vi "State Machine User Manager.vi"() -> ()   [LabVIEW 2024]
doc: "This VI shows how to implement a state machine based, stand-alone user manager using the Easy User Manager package."
uses:
  EasyUserManager/EasyUserManager.lvclass
  <vilib>/regexp/Match Regular Expression.xnode
  Type Definitions/States.ctl
  Type Definitions/Data.ctl
panel:
  in  "Main Tab":T1(tab)=enum."Execution"
  out "Current User":string
  in  "Fill LoginName/Group from Lists":bool=TRUE
  in  "Groups":i32(listbox)=-1
  in  "Tab Control":T2(tab)
  in  "Create Group Button":bool
  in  "Group Name (Create/Delete)":string caption="Group Name"
  in  "Delete Group Button":bool
  in  "Create User Button":bool
  in  "LoginName (Create/Delete)":string caption="LoginName"
  in  "Password (Create)":string caption="Password (only needed for creating)"
  in  "Delete User Button":bool
  in  "New Privilege Value (User Parameters)":bool caption="New Value"
  in  "Privilege (User Configuration)":string caption="Privilege"
  in  "Set Privilege (User Parameters)":bool
  in  "Password (Parameters)":string caption="Password"
  in  "Set Password Button":bool
  in  "Set Full Name (User Parameters)":bool
  in  "Full Name (User Parameters)":string caption="Full Name"
  in  "LoginName (Configuration)":string caption="LoginName"
  in  "Add User to Group Button":bool
  in  "LoginName (Add/Rem User to Group)":string caption="LoginName (User)"
  in  "Group Name (Add/Rem User to Group)":string caption="Group Name"
  in  "Remove User from Group":bool
  in  "Set Group Privilege":bool
  in  "Privilege (Group)":string caption="Privilege"
  in  "New Privilege Value (Group)":bool caption="New Value"
  out "Group Exists Indicator":bool
  out "User Exists Indicator":bool
  in  "Group Exists":bool
  in  "Password (Validation)":string caption="Password"
  in  "LoginName (Validation)":string caption="LoginName"
  in  "Privilege (Validation)":string caption="Privilege"
  in  "Validate Password":bool
  out "Password OK":bool
  in  "Check Privilege":bool
  out "Has privilege":bool
  in  "User Exists":bool
  in  "Users (Groups)":i32(listbox)=-1
  in  "TestStand UI Application Manager":refnum<k7>(container)
  # "Logging in..."
  # "Shutting down..."
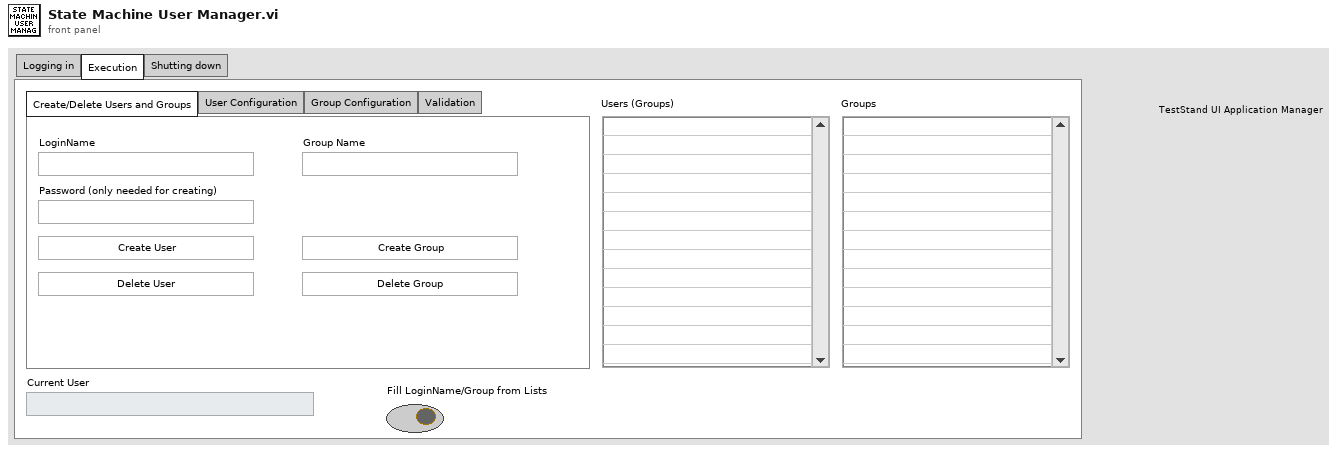
[diagram p1: front panel]
types:
  T1 = enum32{"Logging in", "Execution", "Shutting down"}
  T2 = enum32{"Create/Delete Users and Groups", "User Configuration", "Group Configuration", "Validation"}
  T3 = typedef "Data.ctl" = cluster{"Application Manager":refnum<k7>, "EasyUserManager":refnum<class "EasyUserManager.lvclass">}
  T4 = typedef "States.ctl" = enum16{"Initialize", "Start TS Application", "Wait for Login", "Check User Privilege", "Update User/Group Lists", "Idle", "Error", "Wrong Privileges", "Exit", "Wait for Shutdown", "Pre-Init Check", "Shutdown TS Application"}
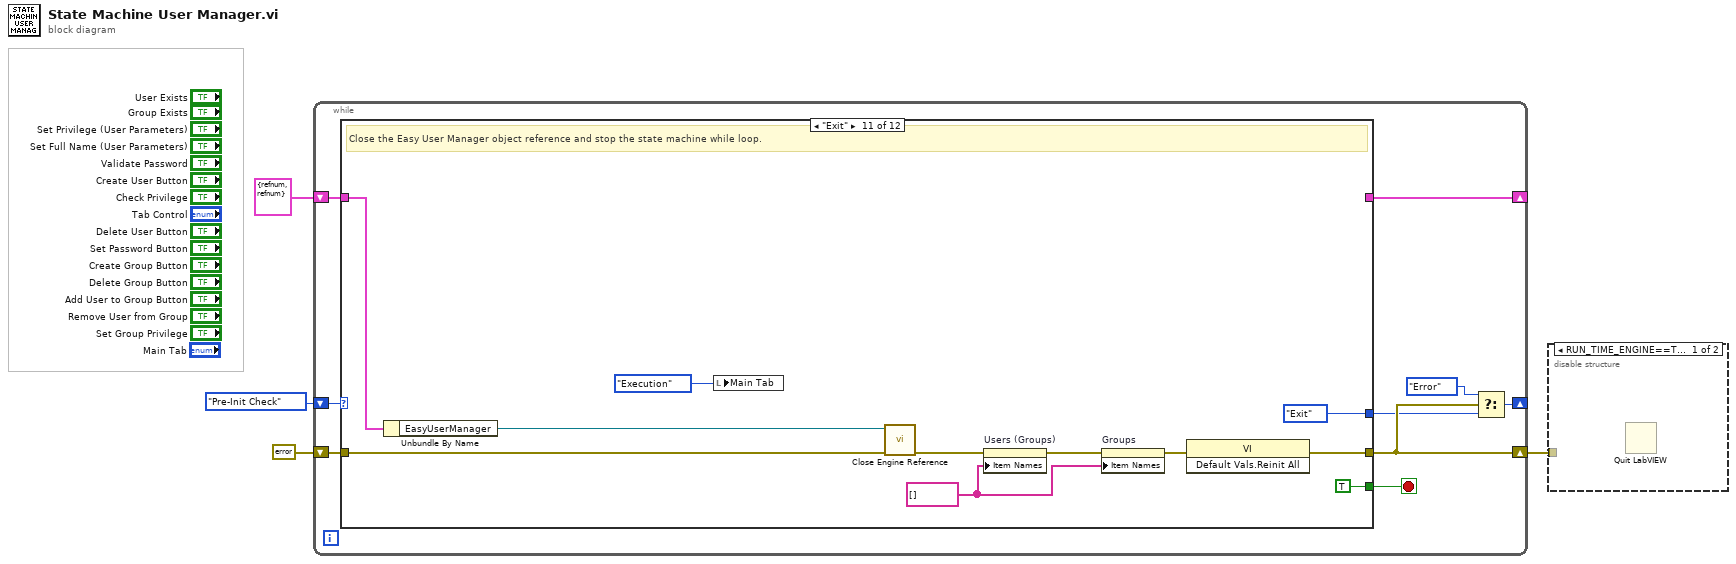
[diagram p0: block diagram]
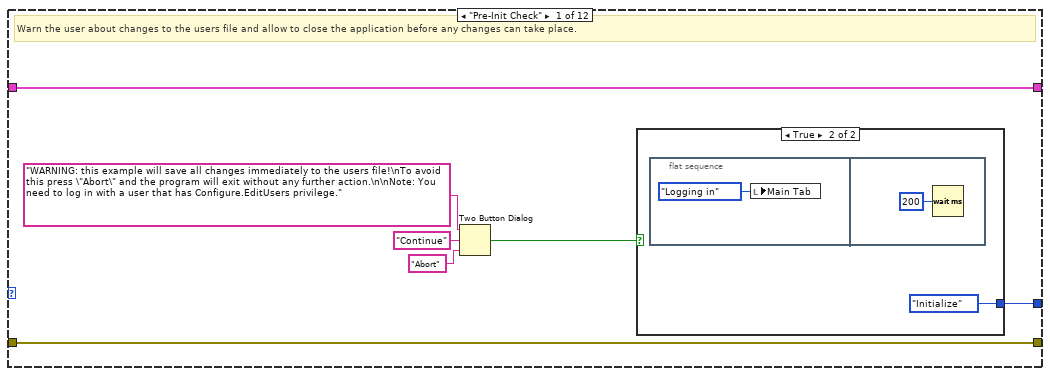
[diagram p3: hidden frame]
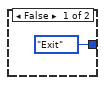
[diagram p4: hidden frame]
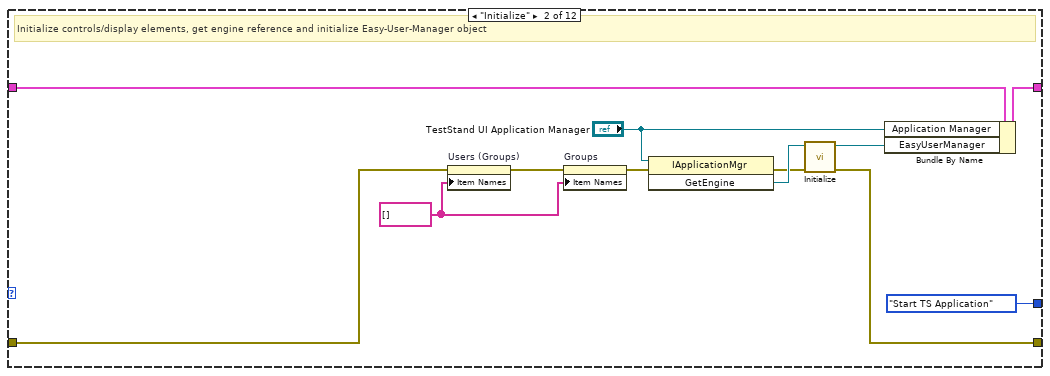
[diagram p5: hidden frame]
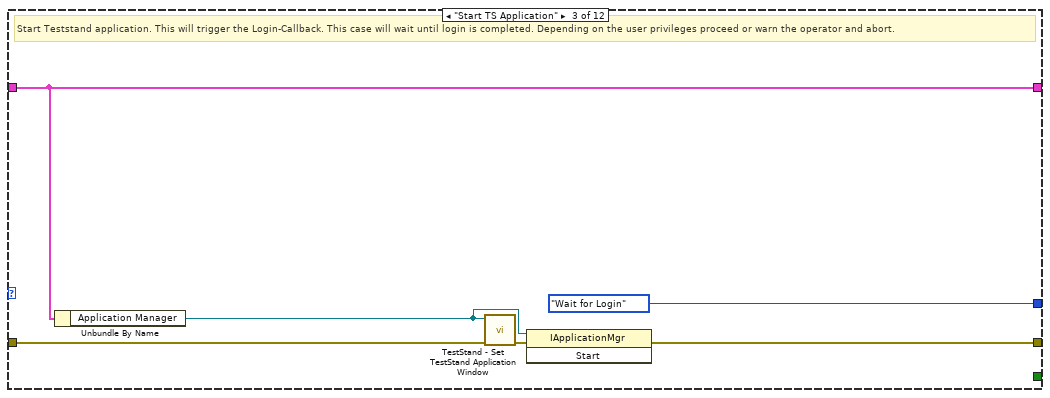
[diagram p6: hidden frame]
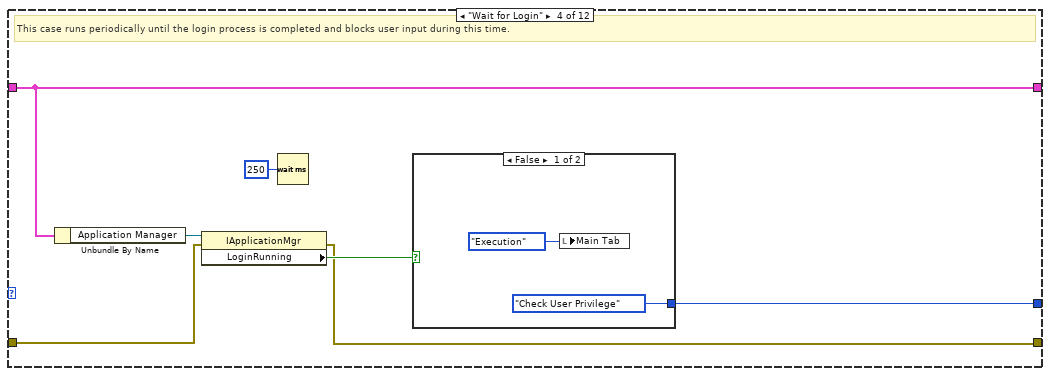
[diagram p7: hidden frame]
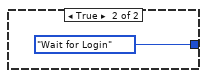
[diagram p8: hidden frame]
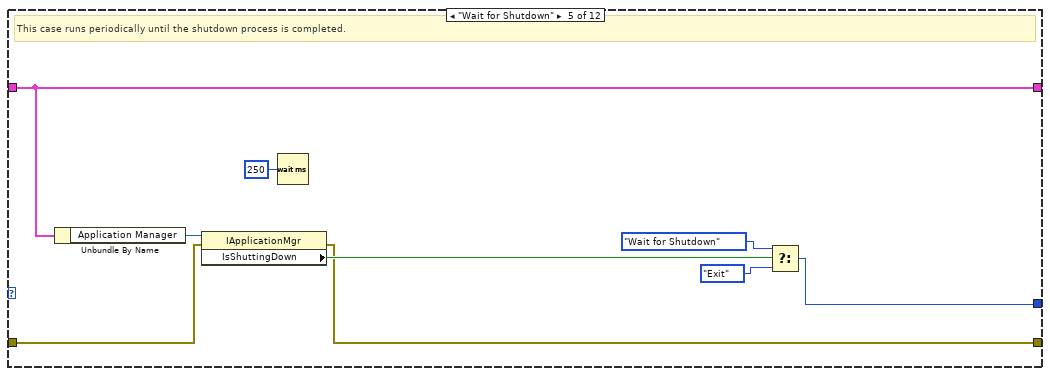
[diagram p9: hidden frame]
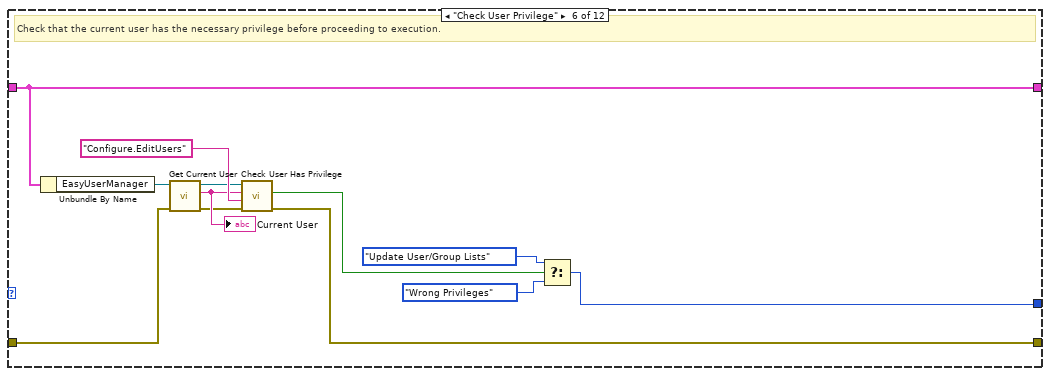
[diagram p10: hidden frame]
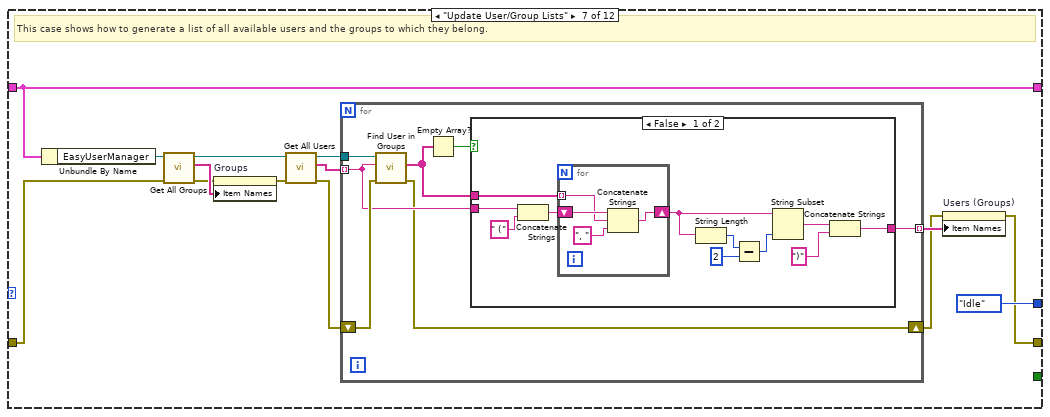
[diagram p11: hidden frame]
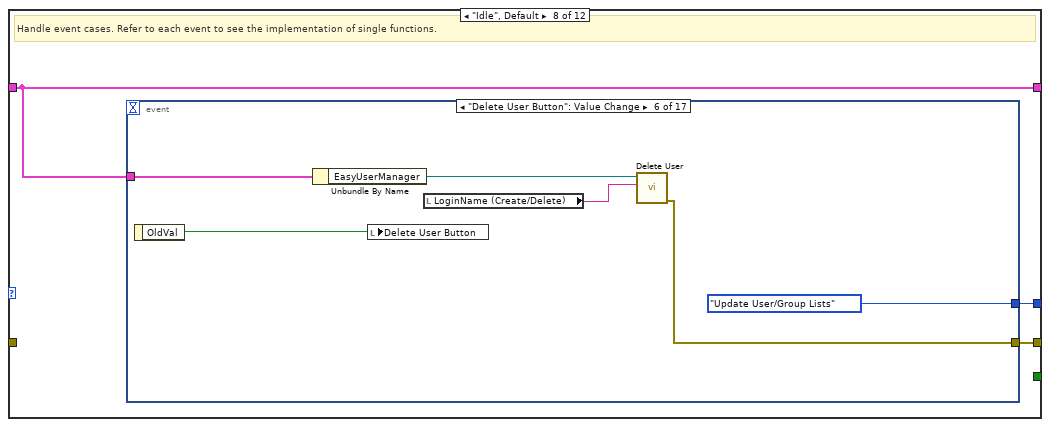
[diagram p13: hidden frame]
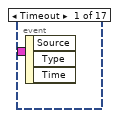
[diagram p14: hidden frame]
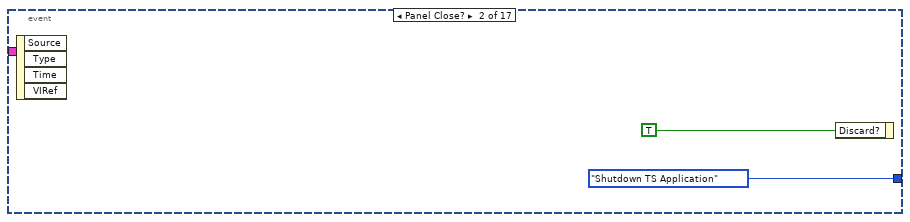
[diagram p15: hidden frame]
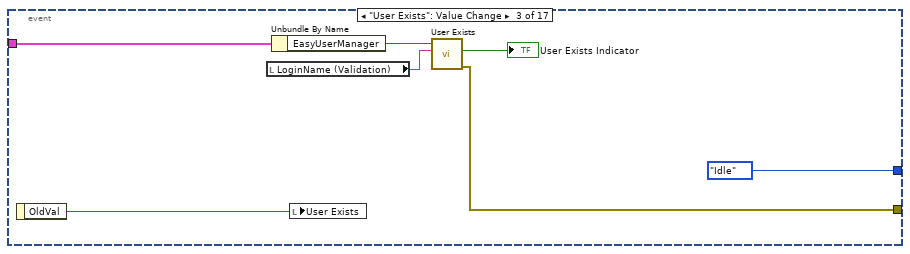
[diagram p16: hidden frame]
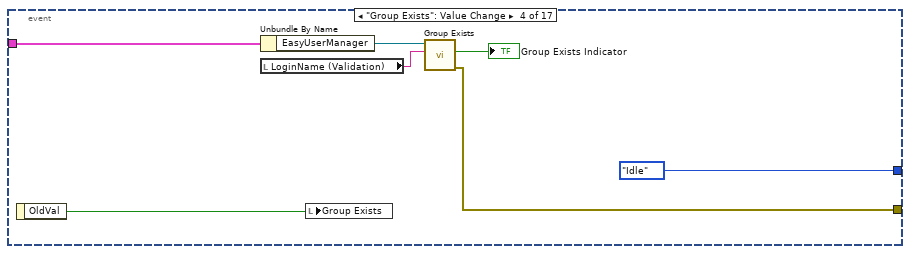
[diagram p17: hidden frame]
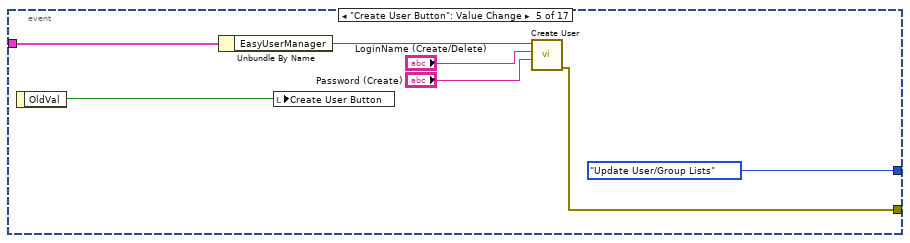
[diagram p18: hidden frame]
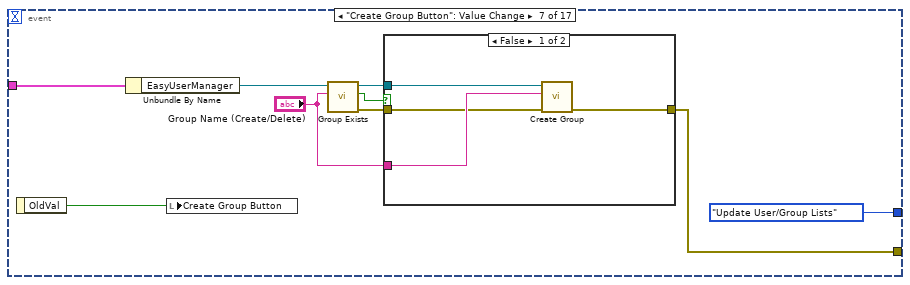
[diagram p19: hidden frame]
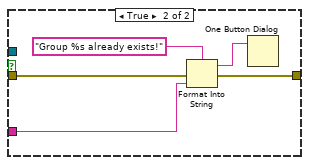
[diagram p20: hidden frame]
diagram:
  n1 = while {
    shift-right: [w6] -> _
    shift-left: States."Pre-Init Check" ("State") -> [w13]
    shift-right: [w5] -> _
    shift-left: T3 {"Application Manager"=refnum, "EasyUserManager"=refnum} ("Data") -> [w11]
    shift-right: [w9] -> w1
    shift-left: errorcluster {"status"=FALSE, "code"=0, "source"=""} ("error constant") -> [w10]
    stop <- w12 stop-if-true
    n2 = case shown="\"Exit\"" w13 {
      tunnel: [_ _ _ _ _ _ _ _ _ _ TRUE _] -> w12
      tunnel: w11 -> [w20 w35 w42 w49 w61 w69 w81 w112 w361 w368 w378 w382]
      tunnel: w10 -> [w16 w25 w37 w46 w58 w64 w74 _ w362 _ w375 w383]
      tunnel: [w16 w26 w38 w43 w53 w68 w82 w111 w358 _ w369 w380] -> w9
      tunnel: [w15 States."Start TS Application" ("State") States."Wait for Login" ("State") w44 w55 w67 States."Idle" ("State") w113 States."Shutdown TS Application" ("State") States."Shutdown TS Application" ("State") States."Exit" ("State") States."Wait for Shutdown" ("State")] -> w7
      tunnel: [w20 w33 w42 w49 w61 w69 w81 w112 w361 w368 _ w382] -> w5
      frame "Pre-Init Check" {
        # "Warn the user about changes to the users file and allow to close the application before any changes can take place."
        n3 = Two Button Dialog(message="WARNING: this example will save all changes immediately to the users file!\nTo avoid this press \"Abort\" and the program will exit without any further action.\n\nNote: You need to log in with a user that has Configure.EditUsers privilege.", 1:"Abort" ("F button name (\"Cancel\")"), 2:"Continue" ("T button name (\"OK\")")) -> (T button?=w14:bool)
        n4 = case shown="True" w14 {
          tunnel: [States."Exit" ("f") States."Initialize" ("State")] -> w15
          frame False {
          }
          frame True {
            n5 = flat-sequence {
              frame #0 {
                n6 = local write "Main Tab"(T1."Logging in" ("Value")) -> ()
              }
              frame #1 {
                n7 = Wait (ms)(milliseconds to wait=u32 200) -> ()  [unwired: 1 out]
              }
            }
          }
        }
      }
      frame "Initialize" {
        w27 = string[] []
        # "Initialize controls/display elements, get engine reference and initialize Easy-User-Manager object"
        n8 = property on="Users (Groups)" class="LstBox (strict)"(error in=w25, "Item Names"=w27) -> (error out=w29:errorcluster)  [unwired: 1 in, 1 out]
        n9 = property on="Groups" class="LstBox (strict)"(error in=w29, "Item Names"=w27) -> (error out=w28:errorcluster)  [unwired: 1 in, 1 out]
        n10 = invoke class="IApplicationMgr" method="GetEngine"(reference="TestStand UI Application Manager", error in=w28) -> (error out=w30:errorcluster, "GetEngine"=w32:refnum<k7>)  [unwired: 1 in, 1 out]
        n11 = call "Initialize.vi"("error in (no error)"=w30, "Engine Reference"=w32) -> ("error out"=w26:errorcluster, "EasyUserManager out"=w31:refnum<class "EasyUserManager.lvclass">)  [unwired: 4 in]
        n12 = Bundle By Name(cluster=w35, "Application Manager"="TestStand UI Application Manager", "EasyUserManager"=w31) -> (w33:T3)
      }
      frame "Start TS Application" {
        # "Start Teststand application. This will trigger the Login-Callback. This case will wait until login is completed. Depending on the user privileges proceed or warn the operator and abort."
        n13 = Unbundle By Name(w42) -> ("Application Manager"=w40:refnum<k7>)
        n14 = call <vilib>:"TestStand - Set TestStand Application Window.vi"("error in (no error)"=w37, "Application Manager"=w40) -> ("error out"=w41:errorcluster)  [unwired: 9 in]
        n15 = invoke class="IApplicationMgr" method="Start"(reference=w40, error in=w41) -> (error out=w38:errorcluster)  [unwired: 1 in, 2 out]
      }
      frame "Wait for Login" {
        # "This case runs periodically until the login process is completed and blocks user input during this time."
        n16 = Unbundle By Name(w49) -> ("Application Manager"=w48:refnum<k7>)
        n17 = property class="IApplicationMgr"(reference=w48, error in=w46) -> (error out=w43:errorcluster, "LoginRunning"=w45:bool)  [unwired: 1 out]
        n18 = Wait (ms)(milliseconds to wait=u32 250) -> ()  [unwired: 1 out]
        n19 = case shown="False" w45 {
          tunnel: [States."Check User Privilege" ("f") States."Wait for Login" ("State")] -> w44
          frame False {
            n20 = local write "Main Tab"(T1."Execution" ("Value")) -> ()
          }
          frame True {
          }
        }
      }
      frame "Wait for Shutdown" {
        # "This case runs periodically until the shutdown process is completed."
        n21 = Unbundle By Name(w61) -> ("Application Manager"=w60:refnum<k7>)
        n22 = property class="IApplicationMgr"(reference=w60, error in=w58) -> (error out=w53:errorcluster, "IsShuttingDown"=w57:bool)  [unwired: 1 out]
        n23 = Wait (ms)(milliseconds to wait=u32 250) -> ()  [unwired: 1 out]
        n24 = Select(t=States."Wait for Shutdown" ("f"), s=w57, f=States."Exit") -> (s? t:f=w55:T4)
      }
      frame "Check User Privilege" {
        # "Check that the current user has the necessary privilege before proceeding to execution."
        n25 = Unbundle By Name(w69) -> ("EasyUserManager"=w66:refnum<class "EasyUserManager.lvclass">)
        n26 = call "Get Current User.vi"("error in (no error)"=w64, "EasyUserManager in"=w66) -> ("error out"=w62:errorcluster, "LoginName"=w63:string, "EasyUserManager out"=w65:refnum<class "EasyUserManager.lvclass">)  [unwired: 3 in]
        "Current User" <- w63
        n27 = call "Check User Has Privilege.vi"("error in (no error)"=w62, "Privilege"="Configure.EditUsers", "LoginName"=w63, "EasyUserManager in"=w65) -> ("error out"=w68:errorcluster, "User Has Privilege"=w73:bool)  [unwired: 1 in, 1 out]
        n28 = Select(t=States."Update User/Group Lists" ("State"), s=w73, f=States."Wrong Privileges") -> (s? t:f=w67:T4)
      }
      frame "Update User/Group Lists" {
        # "This case shows how to generate a list of all available users and the groups to which they belong."
        n29 = Unbundle By Name(w81) -> ("EasyUserManager"=w79:refnum<class "EasyUserManager.lvclass">)
        n30 = call "Get All Groups.vi"("error in (no error)"=w74, "EasyUserManager in"=w79) -> ("error out"=w76:errorcluster, "Groups"=w77:string[], "EasyUserManager out"=w78:refnum<class "EasyUserManager.lvclass">)  [unwired: 3 in]
        n31 = property on="Groups" class="LstBox (strict)"(error in=w76, "Item Names"=w77) -> (error out=w75:errorcluster)  [unwired: 1 in, 1 out]
        n32 = call "Get All Users.vi"("error in (no error)"=w75, "EasyUserManager in"=w78) -> ("error out"=w86:errorcluster, "Users"=w85:string[], "EasyUserManager out"=w80:refnum<class "EasyUserManager.lvclass">)  [unwired: 3 in]
        n33 = for {
          tunnel: w85 -> [w93] mode=indexing
          shift-right: [w92] -> w83
          shift-left: w86 -> [w94]
          tunnel: [w90] -> w84 mode=indexing
          tunnel: w80 -> [w91]
          n34 = call "Find User in Groups.vi"("error in (no error)"=w94, "LoginName"=w93, "EasyUserManager in"=w91) -> ("error out"=w92:errorcluster, "Groups"=w89:string[])  [unwired: 1 in, 2 out]
          n35 = Empty Array?(array=w89) -> (empty?=w88:bool)
          n36 = case shown="False" w88 {
            tunnel: w93 -> [w103 w110]
            tunnel: [w96 w110] -> w90
            tunnel: w89 -> [w95 _]
            frame False {
              n37 = Concatenate Strings(w103, " (" ("string")) -> (w104:string)
              n38 = for {
                tunnel: w95 -> [w108] mode=indexing
                shift-right: [w106] -> w102
                shift-left: w104 -> [w109]
                n39 = Concatenate Strings(w109, w108, ", " ("string")) -> (w106:string)
              }
              n40 = String Length(string=w102) -> (length=w101:i32)
              n41 = Subtract(x=w101, y=2) -> (x-y=w99:i32)
              n42 = String Subset(string=w102, length (rest)=w99) -> (substring=w98:string)  [unwired: 1 in]
              n43 = Concatenate Strings(w98, ")" ("string")) -> (w96:string)
            }
            frame True {
            }
          }
        }
        n44 = property on="Users (Groups)" class="LstBox (strict)"(error in=w83, "Item Names"=w84) -> (error out=w82:errorcluster)  [unwired: 1 in, 1 out]
      }
      frame "Idle", Default {
        # "Handle event cases. Refer to each event to see the implementation of single functions."
        n45 = event shown="[5] \"Delete User Button\": Value Change" {
          selector: _ -> [_ _ _ _ _ _ _ _ _ _ _ _ _ _ _ _ _]
          dyn-events: _ -> [_ _ _ _ _ _ _ _ _ _ _ _ _ _ _ _ _]
          timeout: _ -> [_ _ _ _ _ _ _ _ _ _ _ _ _ _ _ _ _]
          tunnel: [_ States."Shutdown TS Application" ("State") States."Idle" ("State") States."Idle" ("State") States."Update User/Group Lists" ("State") States."Update User/Group Lists" ("State") States."Update User/Group Lists" ("State") States."Update User/Group Lists" ("State") States."Idle" ("State") States."Idle" ("State") States."Idle" ("State") States."Idle" ("State") States."Update User/Group Lists" ("State") States."Update User/Group Lists" ("State") States."Idle" ("State") States."Idle" ("State") States."Idle" ("State")] -> w113
          tunnel: w112 -> [_ _ w121 w128 w135 w141 w150 w165 w171 w181 w187 _ w325 w332 w340 w348 w356]
          tunnel: [_ _ w119 w126 w131 w139 w144 w163 w168 w177 w185 w189 w321 w328 w338 w343 w351] -> w111
          event Timeout {
            n46 = event-data() -> ()  [unwired: 1 in, 3 out]
          }
          event Panel Close? {
            n47 = event-data() -> ()  [unwired: 1 in, 4 out]
            n48 = event-data("Discard?"=TRUE) -> ()  [unwired: 1 in, 1 out]
          }
          event "User Exists": Value Change {
            n49 = event-data() -> ("OldVal"=w122:bool)  [unwired: 1 in]
            n50 = local read "LoginName (Validation)"() -> (w117:string)
            n51 = Unbundle By Name(w121) -> ("EasyUserManager"=w120:refnum<class "EasyUserManager.lvclass">)
            n52 = local write "User Exists"(w122) -> ()
            n53 = call "User Exists.vi"("LoginName"=w117, "EasyUserManager in"=w120) -> ("error out"=w119:errorcluster, "User Exists"=→"User Exists Indicator":bool)  [unwired: 3 in, 1 out]
          }
          event "Group Exists": Value Change {
            n54 = event-data() -> ("OldVal"=w129:bool)  [unwired: 1 in]
            n55 = Unbundle By Name(w128) -> ("EasyUserManager"=w127:refnum<class "EasyUserManager.lvclass">)
            n56 = local read "LoginName (Validation)"() -> (w125:string)
            n57 = local write "Group Exists"(w129) -> ()
            n58 = call "Group Exists.vi"("Group Name"=w125, "EasyUserManager in"=w127) -> ("error out"=w126:errorcluster, "Group Exists"=→"Group Exists Indicator":bool)  [unwired: 3 in, 1 out]
          }
          event "Create User Button": Value Change {
            n59 = event-data() -> ("OldVal"=w136:bool)  [unwired: 1 in]
            n60 = Unbundle By Name(w135) -> ("EasyUserManager"=w134:refnum<class "EasyUserManager.lvclass">)
            n61 = local write "Create User Button"(w136) -> ()
            n62 = call "Create User.vi"("Password"="Password (Create)", "LoginName"="LoginName (Create/Delete)", "EasyUserManager in"=w134) -> ("error out"=w131:errorcluster)  [unwired: 5 in, 1 out]
          }
          event "Delete User Button": Value Change {
            n63 = event-data() -> ("OldVal"=w142:bool)  [unwired: 1 in]
            n64 = Unbundle By Name(w141) -> ("EasyUserManager"=w140:refnum<class "EasyUserManager.lvclass">)
            n65 = local write "Delete User Button"(w142) -> ()
            n66 = local read "LoginName (Create/Delete)"() -> (w138:string)
            n67 = call "Delete User.vi"("LoginName"=w138, "EasyUserManager in"=w140) -> ("error out"=w139:errorcluster)  [unwired: 6 in, 1 out]
          }
          event "Create Group Button": Value Change {
            n68 = event-data() -> ("OldVal"=w151:bool)  [unwired: 1 in]
            n69 = Unbundle By Name(w150) -> ("EasyUserManager"=w145:refnum<class "EasyUserManager.lvclass">)
            n70 = local write "Create Group Button"(w151) -> ()
            n71 = call "Group Exists.vi"("Group Name"="Group Name (Create/Delete)", "EasyUserManager in"=w145) -> ("error out"=w147:errorcluster, "Group Exists"=w146:bool, "EasyUserManager out"=w148:refnum<class "EasyUserManager.lvclass">)  [unwired: 3 in]
            n72 = case shown="False" w146 {
              tunnel: [w155 w159] -> w144
              tunnel: w148 -> [w154 _]
              tunnel: "Group Name (Create/Delete)" -> [w153 w157]
              tunnel: w147 -> [w152 w158]
              frame False {
                n73 = call "Create Group.vi"("error in (no error)"=w152, "Group Name"=w153, "EasyUserManager in"=w154) -> ("error out"=w155:errorcluster)  [unwired: 5 in, 1 out]
              }
              frame True {
                n74 = Format Into String(format string="Group %s already exists!", error in=w158, w157) -> (resulting string=w156:string, error out=w159:errorcluster)  [unwired: 1 in]
                n75 = One Button Dialog(message=w156) -> ()  [unwired: 1 in, 1 out]
              }
            }
          }
          event "Delete Group Button": Value Change {
            n76 = event-data() -> ("OldVal"=w166:bool)  [unwired: 1 in]
            n77 = Unbundle By Name(w165) -> ("EasyUserManager"=w164:refnum<class "EasyUserManager.lvclass">)
            n78 = local read "Group Name (Create/Delete)"() -> (w162:string)
            n79 = local write "Delete Group Button"(w166) -> ()
            n80 = call "Delete Group.vi"("Group Name"=w162, "EasyUserManager in"=w164) -> ("error out"=w163:errorcluster)  [unwired: 6 in, 1 out]
          }
          event "Set Password Button": Value Change {
            n81 = event-data() -> ("OldVal"=w173:bool)  [unwired: 1 in]
            n82 = Unbundle By Name(w171) -> ("EasyUserManager"=w170:refnum<class "EasyUserManager.lvclass">)
            n83 = local write "Set Password Button"(w173) -> ()
            n84 = call "Set User Password.vi"("New Password"="Password (Parameters)", "LoginName"="LoginName (Configuration)", "EasyUserManager in"=w170) -> ("error out"=w168:errorcluster)  [unwired: 5 in, 1 out]
          }
          event "Set Privilege (User Parameters)": Value Change {
            n85 = event-data() -> ("OldVal"=w175:bool)  [unwired: 1 in]
            n86 = local write "Set Privilege (User Parameters)"(w175) -> ()
            n87 = local read "LoginName (Configuration)"() -> (w179:string)
            n88 = Unbundle By Name(w181) -> ("EasyUserManager"=w180:refnum<class "EasyUserManager.lvclass">)
            n89 = call "Set User Privilege.vi"("New Value"="New Privilege Value (User Parameters)", "Privilege"="Privilege (User Configuration)", "LoginName"=w179, "EasyUserManager in"=w180) -> ("error out"=w177:errorcluster)  [unwired: 4 in, 1 out]
          }
          event "Set Full Name (User Parameters)": Value Change {
            n90 = event-data() -> ("OldVal"=w188:bool)  [unwired: 1 in]
            n91 = local read "LoginName (Configuration)"() -> (w184:string)
            n92 = local write "Set Full Name (User Parameters)"(w188) -> ()
            n93 = Unbundle By Name(w187) -> ("EasyUserManager"=w186:refnum<class "EasyUserManager.lvclass">)
            n94 = call "Set User FullName.vi"("FullName"="Full Name (User Parameters)", "LoginName"=w184, "EasyUserManager in"=w186) -> ("error out"=w185:errorcluster)  [unwired: 5 in, 1 out]
          }
          event "Users (Groups)", "Groups": Value Change {
            n95 = event-data() -> ()  [unwired: 1 in, 3 out]
            n96 = case shown="True" "Fill LoginName/Group from Lists" {
              tunnel: [_ w200] -> w189
              frame False {
              }
              frame True {
                n97 = property on="Users (Groups)" class="LstBox (strict)"() -> (error out=w194:errorcluster, "Item Names"=w202:string[])  [unwired: 2 in, 1 out]
                n98 = Index Array(array=w202, index="Users (Groups)") -> (element=w196:string)
                n99 = xnode "Match Regular Expression"("input string"=w196, "regular expression"=" \\(.*\\)", "error in"=w194) -> ("before match"=w192:string, "error out"=w193:errorcluster)  [unwired: 3 in, 3 out]
                n100 = property on="Groups" class="LstBox (strict)"(error in=w193) -> (error out=w200:errorcluster, "Item Names"=w199:string[])  [unwired: 1 in, 1 out]
                n101 = Index Array(array=w199, index="Groups") -> (element=w197:string)
                n102 = local write "Group Name (Create/Delete)"(w197) -> ()
                n103 = local write "Group Name (Add/Rem User to Group)"(w197) -> ()
                n104 = local write "LoginName (Validation)"(w192) -> ()
                n105 = local write "LoginName (Configuration)"(w192) -> ()
                n106 = local write "LoginName (Create/Delete)"(w192) -> ()
                n107 = local write "LoginName (Add/Rem User to Group)"(w192) -> ()
              }
            }
          }
          event "Add User to Group Button": Value Change {
            n108 = event-data() -> ("OldVal"=w326:bool)  [unwired: 1 in]
            n109 = local write "Add User to Group Button"(w326) -> ()
            n110 = Unbundle By Name(w325) -> ("EasyUserManager"=w324:refnum<class "EasyUserManager.lvclass">)
            n111 = call "Add User to Group.vi"("Group Name"="Group Name (Add/Rem User to Group)", "LoginName"="LoginName (Add/Rem User to Group)", "EasyUserManager in"=w324) -> ("error out"=w321:errorcluster)  [unwired: 5 in, 1 out]
          }
          event "Remove User from Group": Value Change {
            n112 = event-data() -> ("OldVal"=w333:bool)  [unwired: 1 in]
            n113 = local write "Remove User from Group"(w333) -> ()
            n114 = local read "Group Name (Add/Rem User to Group)"() -> (w329:string)
            n115 = local read "LoginName (Add/Rem User to Group)"() -> (w330:string)
            n116 = Unbundle By Name(w332) -> ("EasyUserManager"=w331:refnum<class "EasyUserManager.lvclass">)
            n117 = call "Remove User from Group.vi"("Group Name"=w329, "LoginName"=w330, "EasyUserManager in"=w331) -> ("error out"=w328:errorcluster)  [unwired: 5 in, 1 out]
          }
          event "Set Group Privilege": Value Change {
            n118 = event-data() -> ("OldVal"=w341:bool)  [unwired: 1 in]
            n119 = local read "Group Name (Add/Rem User to Group)"() -> (w336:string)
            n120 = local write "Set Group Privilege"(w341) -> ()
            n121 = Unbundle By Name(w340) -> ("EasyUserManager"=w339:refnum<class "EasyUserManager.lvclass">)
            n122 = call "Set Group Privilege.vi"("New Value"="New Privilege Value (Group)", "Privilege"="Privilege (Group)", "Group Name"=w336, "EasyUserManager in"=w339) -> ("error out"=w338:errorcluster)  [unwired: 4 in, 1 out]
          }
          event "Validate Password": Value Change {
            n123 = event-data() -> ("OldVal"=w349:bool)  [unwired: 1 in]
            n124 = Unbundle By Name(w348) -> ("EasyUserManager"=w347:refnum<class "EasyUserManager.lvclass">)
            n125 = local write "Validate Password"(w349) -> ()
            n126 = call "Validate Password.vi"("Password"="Password (Validation)", "LoginName"="LoginName (Validation)", "EasyUserManager in"=w347) -> ("error out"=w343:errorcluster, "Password OK"=→"Password OK":bool)  [unwired: 2 in, 1 out]
          }
          event "Check Privilege": Value Change {
            n127 = event-data() -> ("OldVal"=w357:bool)  [unwired: 1 in]
            n128 = local read "LoginName (Validation)"() -> (w354:string)
            n129 = Unbundle By Name(w356) -> ("EasyUserManager"=w355:refnum<class "EasyUserManager.lvclass">)
            n130 = local write "Check Privilege"(w357) -> ()
            n131 = call "Check User Has Privilege.vi"("Privilege"="Privilege (Validation)", "LoginName"=w354, "EasyUserManager in"=w355) -> ("error out"=w351:errorcluster, "User Has Privilege"=→"Has privilege":bool)  [unwired: 2 in, 1 out]
          }
        }
      }
      frame "Error" {
        # "Error Case: display error to user, then close the application."
        n132 = call <vilib>:"Simple Error Handler.vi"("error in (no error)"=w362) -> ("error out"=w359:errorcluster)  [unwired: 4 in, 4 out]
        n133 = call <vilib>:"Clear Errors.vi"("error in (no error)"=w359) -> ("error out"=w358:errorcluster)  [unwired: 5 in, 1 out]
      }
      frame "Wrong Privileges" {
        # "User does not have the necessary privileges to modify users file. Warn operator and close the application."
        n134 = local read "Current User"() -> (w364:string)
        n135 = Format Into String(format string="User \"%s\" does not have Configure.EditUser privilege!" ("message"), w364) -> (resulting string=w363:string)  [unwired: 2 in, 1 out]
        n136 = One Button Dialog(message=w363, button name ("OK")="Exit") -> ()  [unwired: 1 out]
      }
      frame "Exit" {
        w371 = string[] []
        # "Close the Easy User Manager object reference and stop the state machine while loop."
        n137 = Unbundle By Name(w378) -> ("EasyUserManager"=w377:refnum<class "EasyUserManager.lvclass">)
        n138 = local write "Main Tab"(T1."Execution" ("Value")) -> ()
        n139 = call "Close Engine Reference.vi"("error in (no error)"=w375, "EasyUserManager in"=w377) -> ("error out"=w372:errorcluster)  [unwired: 4 in, 1 out]
        n140 = property on="Users (Groups)" class="LstBox (strict)"(error in=w372, "Item Names"=w371) -> (error out=w373:errorcluster)  [unwired: 1 in, 1 out]
        n141 = property on="Groups" class="LstBox (strict)"(error in=w373, "Item Names"=w371) -> (error out=w370:errorcluster)  [unwired: 1 in, 1 out]
        n142 = invoke class="VI" method="Default Vals.Reinit All"(error in=w370) -> (error out=w369:errorcluster)  [unwired: 2 in, 2 out]
      }
      frame "Shutdown TS Application" {
        # "Shut down the Teststand application. This will trigger the Logout-callback."
        n143 = Unbundle By Name(w382) -> ("Application Manager"=w384:refnum<k7>)
        n144 = invoke class="IApplicationMgr" method="Shutdown"(reference=w384, error in=w383) -> (error out=w380:errorcluster)  [unwired: 1 in, 2 out]
        n145 = flat-sequence {
          frame #0 {
            n146 = local write "Main Tab"(T1."Shutting down" ("Value")) -> ()
          }
          frame #1 {
            n147 = Wait (ms)(milliseconds to wait=u32 200) -> ()  [unwired: 1 out]
          }
        }
      }
    }
    n148 = Select(t=States."Error" ("State"), s=w9, f=w7) -> (s? t:f=w6:T4)
  }
  n149 = disable-structure shown="RUN_TIME_ENGINE==True" {
    disable-tunnel: w1 -> [_ _]
    frame condition #0 {
      n150 = Quit LabVIEW() -> ()  [unwired: 1 in]
    }
    frame condition #1 (active) {
    }
  }
